vi "C_Encode_CAN_to_WS.vi"(6 "brs":bool, 7 "ide":bool, 8 "error in (no error)":errorcluster, 9 "fdf":bool, 10 "id":u32 format="%.0x", 11 "data":u8[](array[numeric]) format="%.0x") -> (0 "error out":errorcluster, 3 "ws frame":u8[](array[numeric]) format="%.0x")   [LabVIEW 2021, in "CANsub_C.lvlib"]
doc: "Encodes one CAN or CAN FD frame into a complete WebSocket frame for the CANsub (serialize + HDLC + WebSocket), ready for TCP Write. Allocates on every call: tests and setup; in the loop use C_Encode_RT."
uses:
  CANsub_C.lvlib
  codec_vis/CANsub_Codec.lvlib
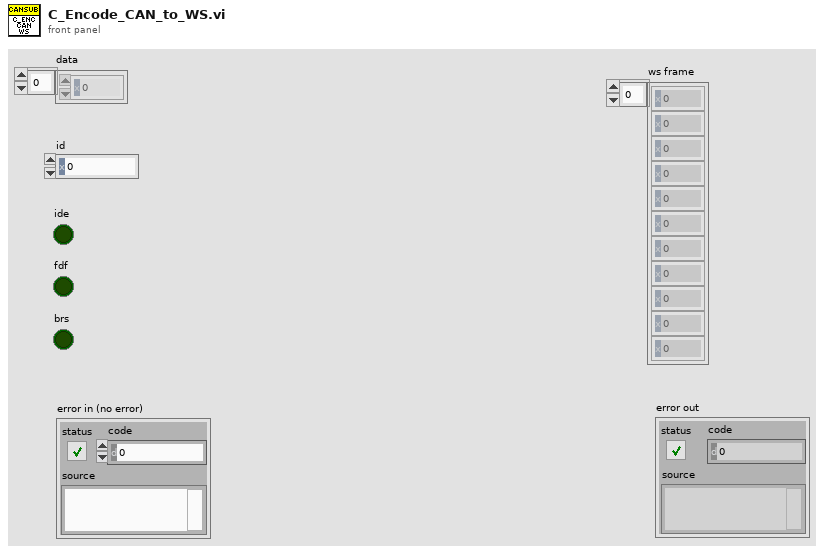
[diagram p1: front panel]
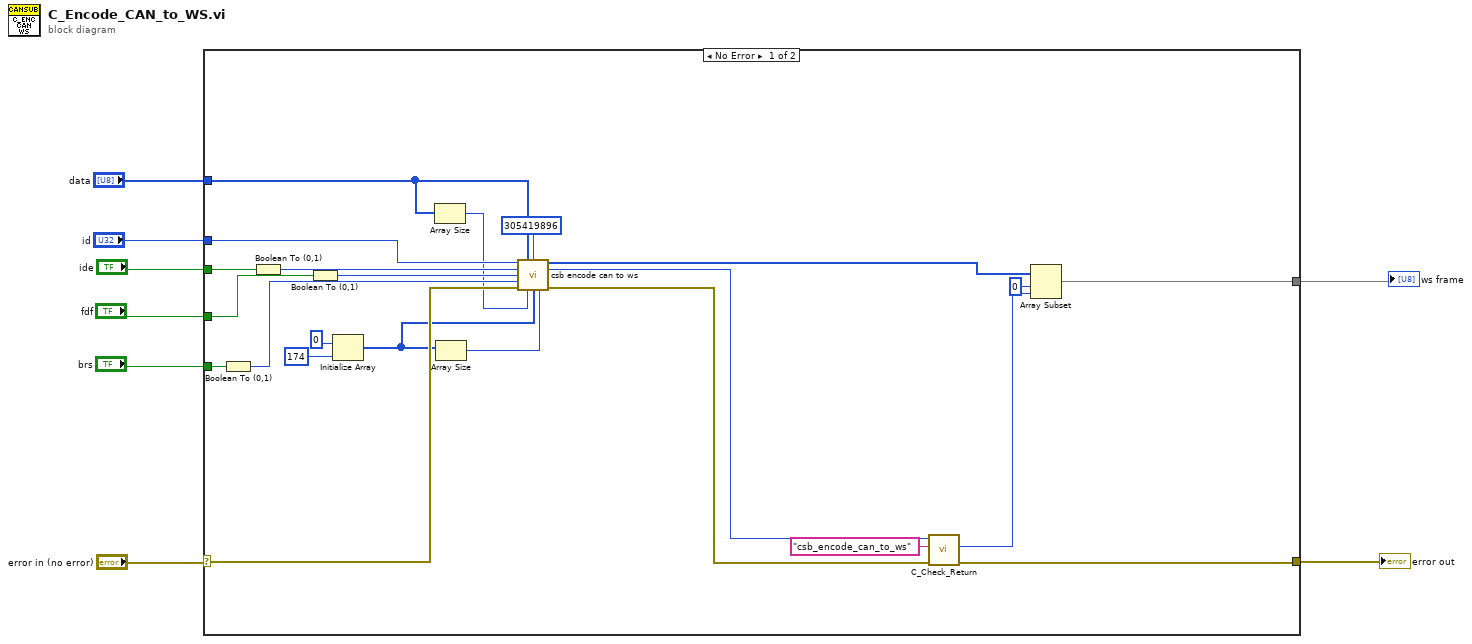
[diagram p0: block diagram]
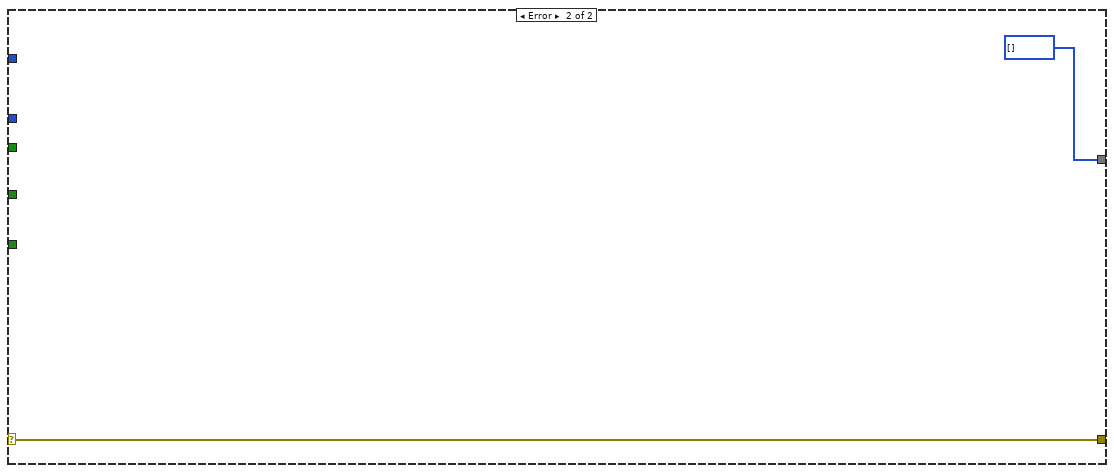
[diagram p2: hidden frame]
diagram:
  n1 = case shown="No Error" "error in (no error)" {
    selector: "error in (no error)" -> [w29 w33]
    tunnel: [w27 w33] -> w7
    tunnel: [w21 u8[] [] ("ws frame")] -> w6
    tunnel: "ide" -> [w20 _]
    tunnel: "fdf" -> [w18 _]
    tunnel: "brs" -> [w16 _]
    tunnel: "id" -> [w14 _]
    tunnel: "data" -> [w10 _]
    frame No Error {
      n2 = Boolean To (0,1)(Boolean=w16) -> (0, 1=w15:i16)
      n3 = Boolean To (0,1)(Boolean=w20) -> (0, 1=w19:i16)
      n4 = Boolean To (0,1)(Boolean=w18) -> (0, 1=w17:i16)
      n5 = Initialize Array(u8 0, 174 ("dimension size")) -> (w11:u8[])
      n6 = Array Size(array=w10) -> (size(s)=w9:i32)
      n7 = Array Size(array=w11) -> (size(s)=w12:i32)
      n8 = call "csb encode can to ws.vi"("id"=w14, "data"=w10, "mask"=u32 305419896, "out_cap"=w12, "ide"=w19, "fdf"=w17, "brs"=w15, "error in (no error)"=w29, "len"=w9, "out"=w11) -> ("out out"=w22:u8[], "function return"=w26:i32, "error out"=w28:errorcluster)  [unwired: 3 in]
      n9 = call "C_Check_Return.vi"("error in (no error)"=w28, "function name"="csb_encode_can_to_ws", "function return"=w26) -> ("error out"=w27:errorcluster, "length"=w24:i32)  [unwired: 6 in, 1 out]
      n10 = Array Subset(array=w22, index=0, length=w24) -> (w21:u8[])
    }
    frame Error {
    }
  }
  "error out" <- w7
  "ws frame" <- w6
